vi "Get Data.vi"(8 "Name":string) -> (3 "Auto":T5)   [LabVIEW 2023]
uses:
  bordeaux-main/Bordeaux/Types/Single Cmd Info.ctl
  <vilib>/picture/picture.llb/imagedata.ctl
  bordeaux-main/Bordeaux/Types/Trajectory Data.ctl
  bordeaux-main/Bordeaux/Types/Segment Type.ctl
panel:
  in  "Path":path=path "/home/lvuser/natinst/bin/Paths"
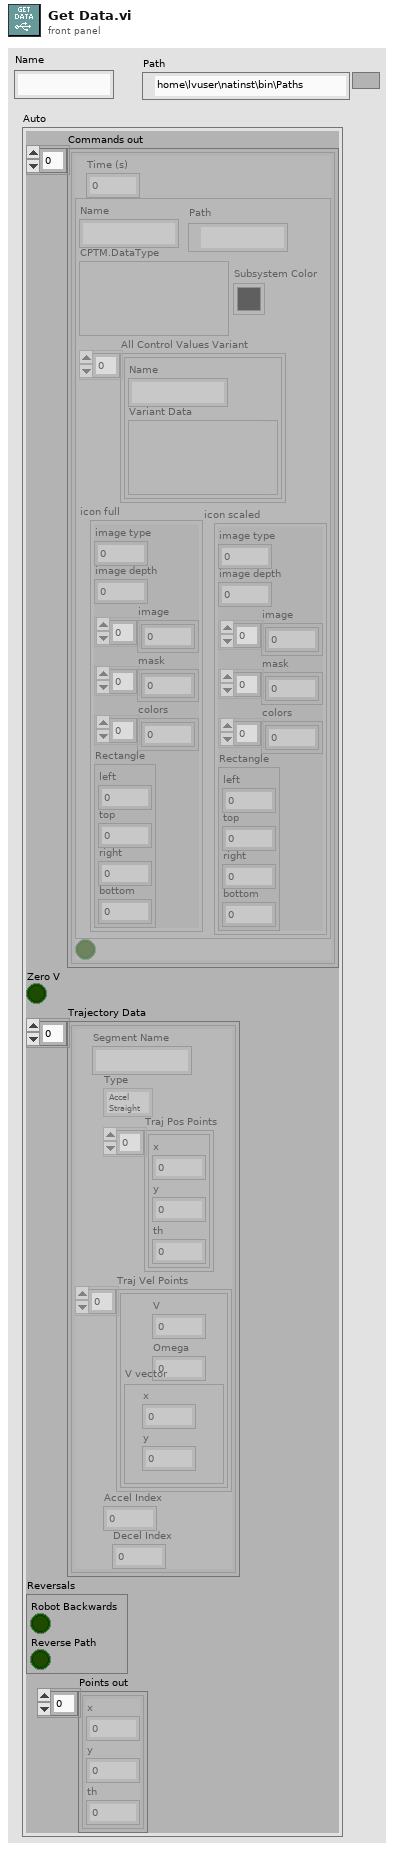
[diagram p1: front panel]
types:
  T1 = typedef "Single Cmd Info.ctl" = cluster{"Name":string, "CPTM.DataType":variant, "All Control Values Variant":cluster{"Name":string, "Variant Data":variant}[], "icon full":T2, "icon scaled":T2, "Path":path, "Subsystem Color":u32}
  T2 = typedef "imagedata.ctl" = cluster{"image type":i32, "image depth":i32, "image":u8[], "mask":u8[], "colors":u32[], "Rectangle":cluster{"left":i16, "top":i16, "right":i16, "bottom":i16}}
  T3 = typedef "Trajectory Data.ctl" = cluster{"Segment Name":string, "Type":T4, "Traj Pos Points":cluster{"x":dbl, "y":dbl, "th":dbl}[], "Traj Vel Points":cluster{"V":dbl, "Omega":dbl, "V vector":cluster{"y":dbl, "x":dbl}}[], "Accel Index":i32, "Decel Index":i32}[]
  T4 = typedef "Segment Type.ctl" = enum16{"Accel Straight", "Const Straight", "Blend", "Circle", "Bezier"}
  T5 = cluster{"Commands out":cluster{"Time (s)":dbl, T1, bool}[], "Zero V":bool, "Trajectory Data":T3, "Reversals":cluster{"Robot Backwards":bool, "Reverse Path":bool}, "Points out":cluster{"x":dbl, "y":dbl, "th":dbl}[]}
  T6 = cluster{"Robot Backwards":bool, "Reverse Path":bool}
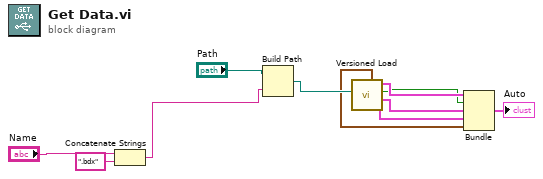
[diagram p0: block diagram]
diagram:
  n1 = Concatenate Strings("Name", ".bdx" ("string")) -> (w2:string)
  n2 = Build Path(base path="Path", name or relative path=w2) -> (appended path=w11:path)
  n3 = call "Versioned Load.vi"("path"=w11) -> ("Reversals"=w7:T6, "Trajectory Data"=w8:T3, "Zero V"=w9:bool, "Commands out"=w10:cluster{"Time (s)":dbl, T1, bool}[], "Points out"=w6:cluster{"x":dbl, "y":dbl, "th":dbl}[])  [unwired: 3 in, 3 out]
  n4 = Bundle("Commands out"=w10, "Zero V"=w9, "Trajectory Data"=w8, "Reversals"=w7, "Points out"=w6) -> (→"Auto":T5)  [unwired: 1 in]
